vi "Close.vi"(1 "Session_id":u32, 2 "UCI_DllPath":path) -> (0 "ResultDescription":string)   [LabVIEW 2015]
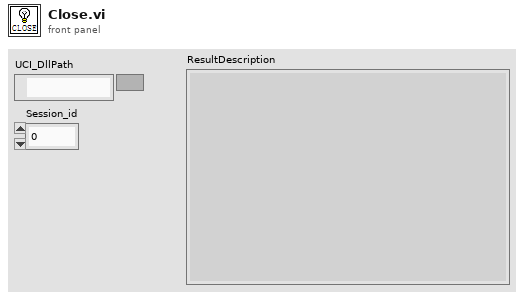
[diagram p1: front panel]
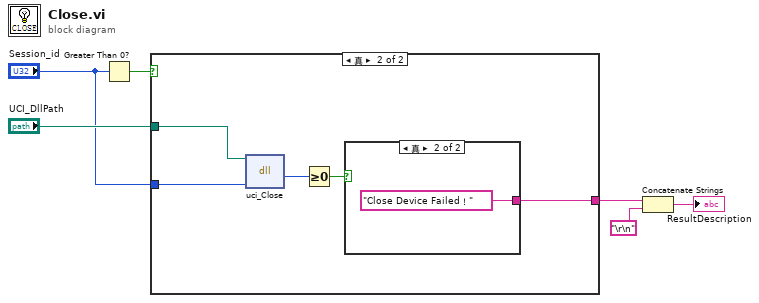
[diagram p0: block diagram]
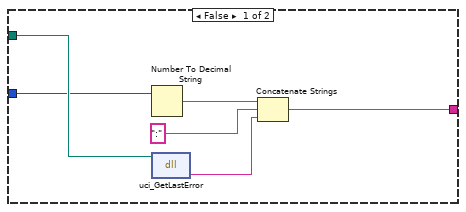
[diagram p2: hidden frame]
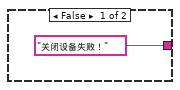
[diagram p3: hidden frame]
diagram:
  n1 = Greater Than 0?(x="Session_id") -> (x > 0?=w6:bool)
  n2 = case shown="真" w6 {
    tunnel: "Session_id" -> [w8 w17]
    tunnel: "UCI_DllPath" -> [w9 w16]
    tunnel: [w7 w13] -> w2
    frame False {
      n3 = Number To Decimal String(number=w8) -> (decimal integer string=w12:string)  [unwired: 1 in]
      n4 = dll-call lib="E:/JL-Project/LabView-Project/ASCII/uci.dll" fn="uci_GetLastError"(path in=w9) -> ("返回类型"=w10:string)  [unwired: 2 in, 2 out]
      n5 = Concatenate Strings(w12, ":" ("字符串"), w10) -> (w7:string)
    }
    frame True {
      n6 = dll-call lib="E:/JL-Project/LabView-Project/ASCII/uci.dll" fn="uci_Close"(path in=w16, "session"=w17) -> ("返回类型"=w15:i32)  [unwired: 3 in, 2 out]
      n7 = Greater Or Equal To 0?(x=w15) -> (x >= 0?=w14:bool)
      n8 = case shown="真" w14 {
        tunnel: ["关闭设备失败！" "Close Device Failed！"] -> w13
        frame False {
        }
        frame True {
        }
      }
    }
  }
  n9 = Concatenate Strings(w2, "\r\n") -> (→"ResultDescription":string)
